vi "Path to absolute path.vi"(4 "path":path) -> (1 "absolute path":path)   [LabVIEW 2021]
doc: "::: CalcExpress Toolkit :::\nCopyright (c) 2000-2026 Konstantin Shifershteyn. All rights reserved."
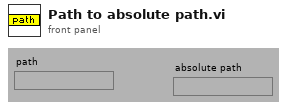
[diagram p1: front panel]
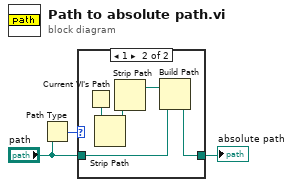
[diagram p0: block diagram]
diagram:
  n1 = Path Type(1:"path") -> (0:w3:i16)
  n2 = case shown="1" w3 {
    tunnel: "path" -> [w4 w6]
    tunnel: [w4 w5] -> w1
    frame 0, Default {
    }
    frame 1 {
      n3 = Current VI's Path() -> (path=w9:path)
      n4 = Strip Path(path=w9) -> (stripped path=w8:path)  [unwired: 1 out]
      n5 = Strip Path(path=w8) -> (stripped path=w7:path)  [unwired: 1 out]
      n6 = Build Path(base path=w7, name or relative path=w6) -> (appended path=w5:path)
    }
  }
  "absolute path" <- w1
